vi "LogInfo2txt.vi"(5 "type":enum16{"txt", "bin"}(ring), 7 "File ID":string, 8 "error in (no error)":errorcluster, 11 "text":string) -> ()   [LabVIEW 2023, in "LoggingProber.lvlib"]
uses:
  LoggingProber.lvlib
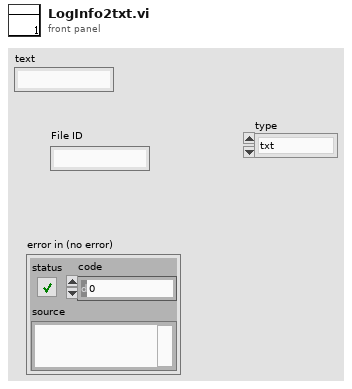
[diagram p1: front panel]
types:
  T1 = enum16{"open", "replace", "create", "open or create", "replace or create", "replace or create with confirmation"}
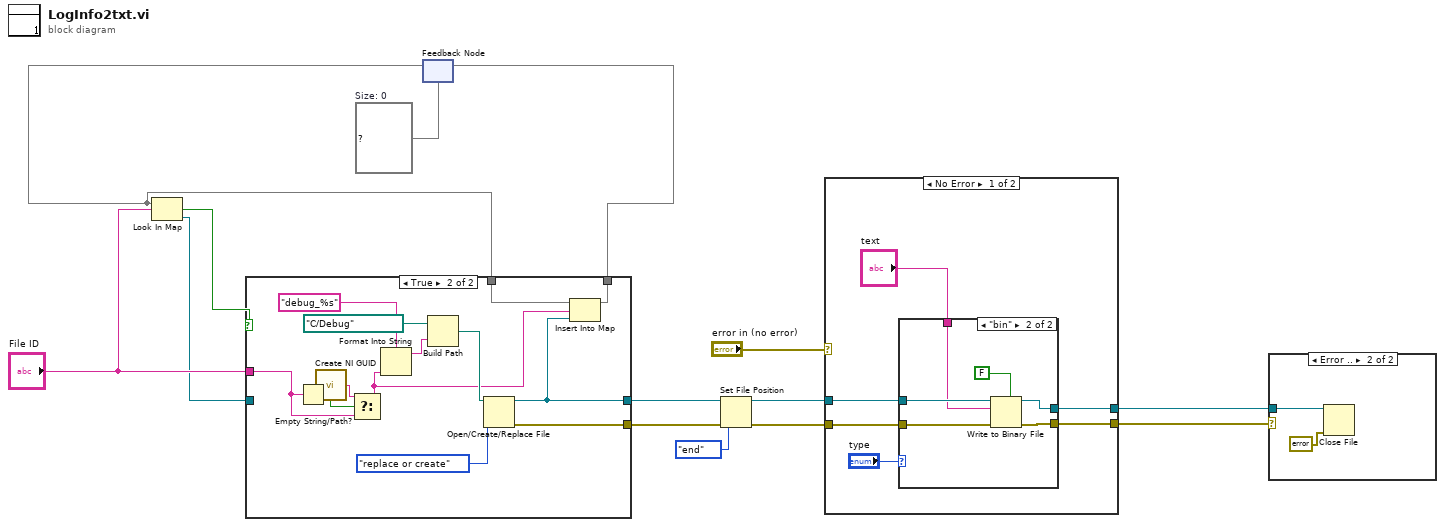
[diagram p0: block diagram]
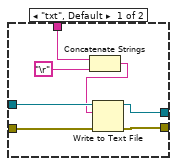
[diagram p2: hidden frame]
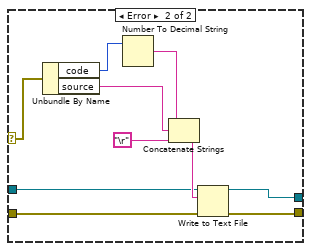
[diagram p3: hidden frame]
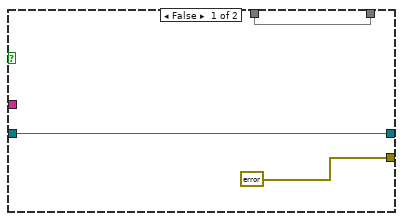
[diagram p4: hidden frame]
diagram:
  w2 = map{string, refnum<file>} {}  # Size: 0
  n1 = feedback #1(w2) -> (w5:map{string, refnum<file>})
  n2 = Look In Map(map=w5, key="File ID") -> (key not found?=w4:bool, value=w3:refnum<file>)  [unwired: 1 in]
  n3 = case shown="True" w4 {
    tunnel: [w17 w19] -> w7
    tunnel: [errorcluster {"status"=FALSE, "code"=0, "source"=""} ("error out") w30] -> w10
    tunnel: w3 -> [w17 _]
    tunnel: "File ID" -> [_ w22]
    tunnel: w5 -> [w15 w21]
    tunnel: [w15 w18] -> w6
    frame False {
    }
    frame True {
      n4 = Empty String/Path?(string/path=w22) -> (empty?=w24:bool)
      n5 = call <vilib>:"Create NI GUID.vi"() -> ("NI GUID"=w23:string)
      n6 = Select(t=w23, s=w24, f=w22) -> (s? t:f=w20:string)
      n7 = Format Into String(format string="debug_%s", w20) -> (resulting string=w26:string)  [unwired: 2 in, 1 out]
      n8 = Build Path(base path=path "C:/Debug" ("file path (use dialog)"), name or relative path=w26) -> (appended path=w28:path)
      n9 = Open/Create/Replace File(file path (use dialog)=w28, operation (0:open)=T1."replace or create") -> (refnum out=w19:refnum<file>, error out=w30:errorcluster)  [unwired: 4 in, 1 out]
      n10 = Insert Into Map(map in=w21, key=w20, value=w19) -> (map out=w18:map{string, refnum<file>})  [unwired: 2 out]
    }
  }
  n11 = feedback-in #1(w6) -> ()
  n12 = Set File Position(refnum=w7, from (0:start)=enum16{"start", "end", "current"}."end", error in=w10) -> (refnum out=w11:refnum<file>, error out=w9:errorcluster)  [unwired: 1 in]
  n13 = case shown="No Error" "error in (no error)" {
    selector: "error in (no error)" -> [_ w54]
    tunnel: [w36 w56] -> w14
    tunnel: [w35 w55] -> w13
    tunnel: w11 -> [w34 w50]
    tunnel: w9 -> [w33 w57]
    frame No Error {
      n14 = case shown="\"bin\"" "type" {
        tunnel: [w43 w46] -> w36
        tunnel: [w42 w48] -> w35
        tunnel: w34 -> [w41 w49]
        tunnel: w33 -> [w40 w47]
        tunnel: "text" -> [w39 w45]
        frame "txt", Default {
          n15 = Concatenate Strings(w39, "\r") -> (w37:string)
          n16 = Write to Text File(file (use dialog)=w41, text=w37, error in=w40) -> (refnum out=w42:refnum<file>, error out=w43:errorcluster)  [unwired: 1 in, 1 out]
        }
        frame "bin" {
          n17 = Write to Binary File(file (use dialog)=w49, data=w45, error in=w47, 5:FALSE ("prepend array or string size? (T)")) -> (refnum out=w48:refnum<file>, error out=w46:errorcluster)  [unwired: 2 in, 1 out]
        }
      }
    }
    frame Error {
      n18 = Unbundle By Name(w54) -> ("code"=w52:i32, "source"=w53:string)
      n19 = Number To Decimal String(number=w52) -> (decimal integer string=w51:string)  [unwired: 1 in]
      n20 = Concatenate Strings(w51, w53, "\r") -> (w58:string)
      n21 = Write to Text File(file (use dialog)=w50, text=w58, error in=w57) -> (refnum out=w55:refnum<file>, error out=w56:errorcluster)  [unwired: 1 in, 1 out]
    }
  }
  n22 = case shown="Error .." w14 {
    tunnel: w13 -> [_ w60]
    frame No Error {
    }
    frame Error {
      n23 = Close File(refnum=w60, error in=errorcluster {"status"=FALSE, "code"=0, "source"=""}) -> ()  [unwired: 2 out]
    }
  }
